vi "SID_oscillator.vi"(5 "sampling info":cluster{"Fs":dbl, "#s":i32}={"Fs"=44100.0, "#s"=50}, 6 "MSB in":bool, 7 "Reg":T1, 9 "reset phase":bool=TRUE) -> (2 "MSB out":bool, 3 "wave":dbl[](array[numeric]))   [LabVIEW 2018]
uses:
  SID_voice_reg.ctl
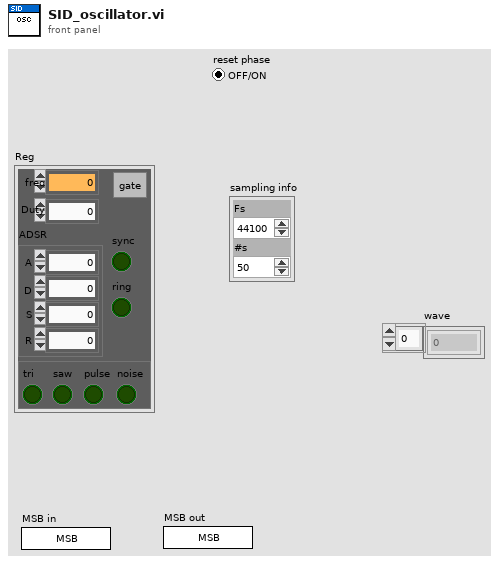
[diagram p1: front panel]
types:
  T1 = typedef "SID_voice_reg.ctl" = cluster{"freq":dbl, "gate":bool, "ADSR":cluster{"A":dbl, "D":dbl, "S":dbl, "R":dbl}, "Duty":dbl, "osc enab":cluster{"tri":bool, "saw":bool, "pulse":bool, "noise":bool}, "sync":bool, "ring":bool}
  T2 = cluster{"tri":bool, "saw":bool, "pulse":bool, "noise":bool}
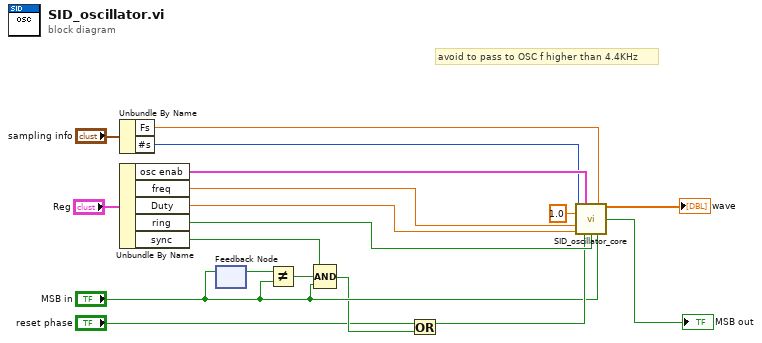
[diagram p0: block diagram]
diagram:
  # "avoid to pass to OSC f higher than 4.4KHz"
  n1 = Unbundle By Name("sampling info") -> ("Fs"=w14:dbl, "#s"=w15:i32)
  n2 = Unbundle By Name("Reg") -> ("osc enab"=w16:T2, "freq"=w1:dbl, "Duty"=w2:dbl, "ring"=w11:bool, "sync"=w5:bool)
  n3 = feedback-in #1("MSB in") -> ()
  n4 = feedback #1() -> (w8:bool)  [unwired: 1 in]
  n5 = Not Equal?(x=w8, y="MSB in") -> (x != y?=w7:bool)
  n6 = Compound Arithmetic op=AND(w5, w7, "MSB in") -> (w4:bool)
  n7 = Or(x="reset phase", y=w4) -> (x .or. y?=w9:bool)
  n8 = call "SID_oscillator_core.vi"("samples"=w15, "wave enab"=w16, "Fs"=w14, "amplitude"=1.0, "freq"=w1, "pulse width"=w2, "reset"=w9, "use ext OSC"=w11, "MSB in"="MSB in") -> ("wave"=→"wave":dbl[], "MSB out"=→"MSB out":bool)  [unwired: 4 in, 1 out]
